vi "Calculate Vector Data.vi"(6 "Data In":T1, 8 "Display State In":T2 caption="State", 9 "X or Magnitude In":waveform(dbl), 10 "Y or Phase In":waveform(dbl), 11 "Order In":u16) -> (4 "Data Out":T1, 5 "R,Theta or X,Y Points Out":cluster{dbl, dbl}[](array[cluster]))   [LabVIEW 2012, in "Vector Function Generator.xctl"]
doc: "Based on the XControl's state, takes the two waveforms as eith R,theta or X,Y data and calculates a complex number waveform from the result/"
uses:
  Vector Function Generator.xctl
  Vector State.ctl
  Vector Data.ctl
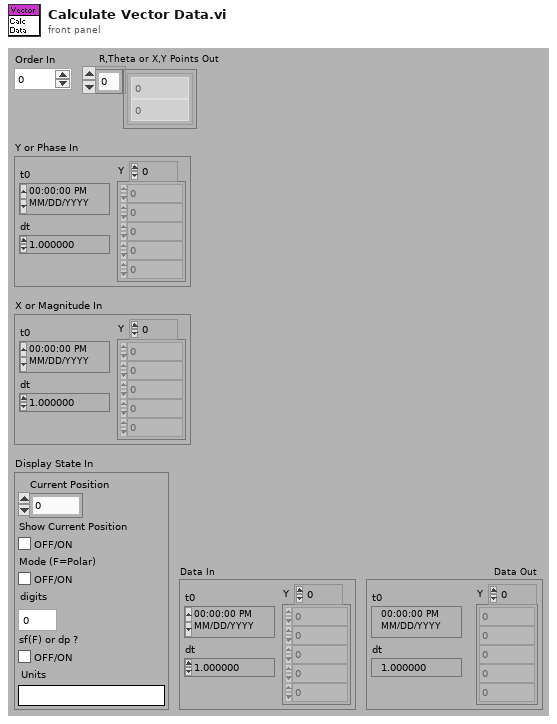
[diagram p1: front panel]
types:
  T1 = typedef "Vector Function Generator.xctl/Vector Data.ctl" = waveform(cdb)
  T2 = typedef "Vector Function Generator.xctl/Vector State.ctl" = cluster{"Current Position":i32, "Show Current Position":bool, "Mode (F=Polar)":bool, "digits":i32, "sf(F) or dp ?":bool, "Units":string}
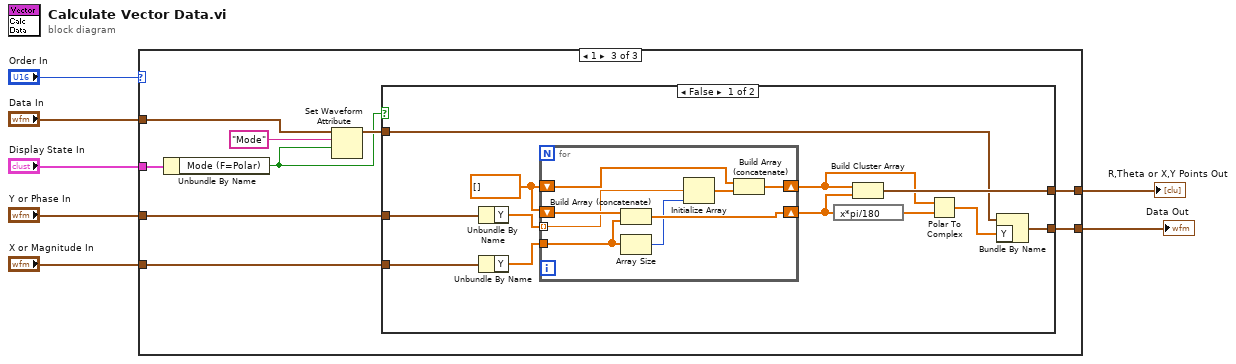
[diagram p0: block diagram]
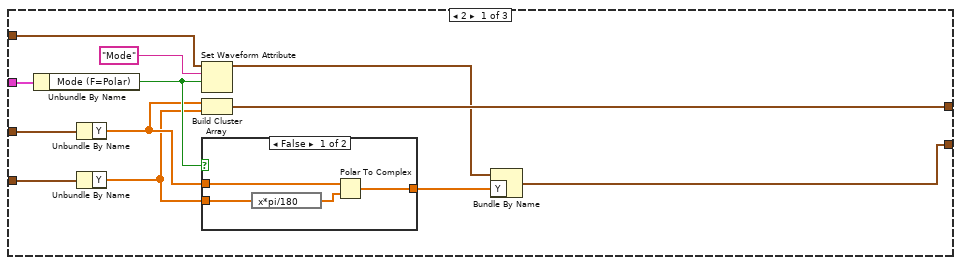
[diagram p2: hidden frame]
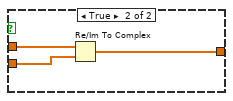
[diagram p3: hidden frame]
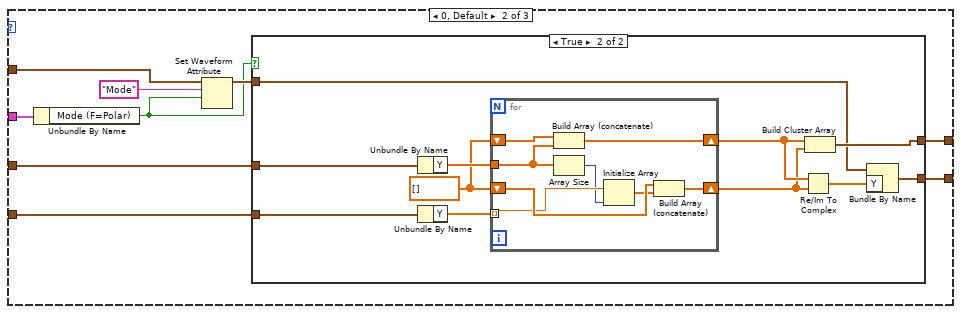
[diagram p4: hidden frame]
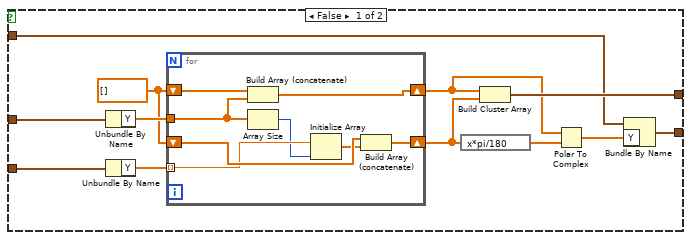
[diagram p5: hidden frame]
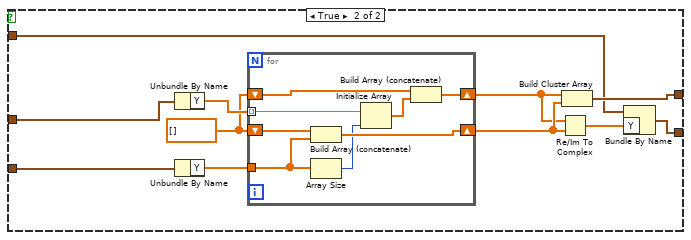
[diagram p6: hidden frame]
diagram:
  n1 = case shown="1" "Order In" {
    tunnel: [w19 w35 w83] -> w6
    tunnel: "Y or Phase In" -> [w18 w34 w82]
    tunnel: "X or Magnitude In" -> [w17 w31 w79]
    tunnel: "Data In" -> [w15 w32 w80]
    tunnel: [w12 w33 w81] -> w5
    tunnel: "Display State In" -> [w13 w30 w78]
    frame 2 {
      n2 = Unbundle By Name(w13) -> ("Mode (F=Polar)"=w11:bool)
      n3 = Unbundle By Name(w18) -> ("Y"=w10:dbl[])
      n4 = Unbundle By Name(w17) -> ("Y"=w9:dbl[])
      n5 = Set Waveform Attribute(5:w11, 6:"Mode" ("name"), 7:w15) -> (3:w14:T1)  [unwired: 1 in, 2 out]
      n6 = Build Cluster Array(w10, w9) -> (w19:cluster{dbl, dbl}[])
      n7 = case shown="False" w11 {
        tunnel: w10 -> [w23 w26]
        tunnel: w9 -> [w22 w25]
        tunnel: [w21 w24] -> w8
        frame False {
          n8 = expression code="x*pi/180"(w22) -> (w20:dbl[])
          n9 = Polar To Complex(1:w20, 2:w23) -> (0:w21:cdb[])
        }
        frame True {
          n10 = Re/Im To Complex(1:w25, 2:w26) -> (0:w24:cdb[])
        }
      }
      n11 = Bundle By Name(cluster=w14, "Y"=w8) -> (w12:T1)
    }
    frame 0, Default {
      n12 = Unbundle By Name(w30) -> ("Mode (F=Polar)"=w28:bool)
      n13 = Set Waveform Attribute(5:w28, 6:"Mode" ("name"), 7:w32) -> (3:w29:T1)  [unwired: 1 in, 2 out]
      n14 = case shown="True" w28 {
        tunnel: [w47 w66] -> w35
        tunnel: w34 -> [w46 w65]
        tunnel: [w38 w59] -> w33
        tunnel: w29 -> [w41 w63]
        tunnel: w31 -> [w43 w61]
        frame False {
          w44 = dbl[] []
          n15 = Unbundle By Name(w46) -> ("Y"=w45:dbl[])
          n16 = Unbundle By Name(w43) -> ("Y"=w42:dbl[])
          n17 = for {
            tunnel: w45 -> [w51]
            shift-right: [w55] -> w40
            shift-left: w44 -> [w54]
            shift-right: [w53] -> w37
            shift-left: w44 -> [w52]
            tunnel: w42 -> [w50] mode=indexing
            n18 = Build Array (concatenate)(w54, w51) -> (w55:dbl[])
            n19 = Array Size(array=w51) -> (size(s)=w49:i32)
            n20 = Initialize Array(w50, w49) -> (w48:dbl[])
            n21 = Build Array (concatenate)(w52, w48) -> (w53:dbl[])
          }
          n22 = expression code="x*pi/180"(w37) -> (w36:dbl[])
          n23 = Build Cluster Array(w40, w37) -> (w47:cluster{dbl, dbl}[])
          n24 = Polar To Complex(1:w36, 2:w40) -> (0:w39:cdb[])
          n25 = Bundle By Name(cluster=w41, "Y"=w39) -> (w38:T1)
        }
        frame True {
          w62 = dbl[] []
          n26 = Unbundle By Name(w65) -> ("Y"=w64:dbl[])
          n27 = Unbundle By Name(w61) -> ("Y"=w60:dbl[])
          n28 = for {
            tunnel: w64 -> [w70]
            shift-right: [w74] -> w58
            shift-left: w62 -> [w73]
            shift-right: [w72] -> w57
            shift-left: w62 -> [w71]
            tunnel: w60 -> [w69] mode=indexing
            n29 = Build Array (concatenate)(w73, w70) -> (w74:dbl[])
            n30 = Array Size(array=w70) -> (size(s)=w68:i32)
            n31 = Initialize Array(w69, w68) -> (w67:dbl[])
            n32 = Build Array (concatenate)(w71, w67) -> (w72:dbl[])
          }
          n33 = Re/Im To Complex(1:w57, 2:w58) -> (0:w56:cdb[])
          n34 = Build Cluster Array(w58, w57) -> (w66:cluster{dbl, dbl}[])
          n35 = Bundle By Name(cluster=w63, "Y"=w56) -> (w59:T1)
        }
      }
    }
    frame 1 {
      n36 = Unbundle By Name(w78) -> ("Mode (F=Polar)"=w76:bool)
      n37 = Set Waveform Attribute(5:w76, 6:"Mode" ("name"), 7:w80) -> (3:w77:T1)  [unwired: 1 in, 2 out]
      n38 = case shown="False" w76 {
        tunnel: [w95 w114] -> w83
        tunnel: w82 -> [w94 w113]
        tunnel: [w86 w107] -> w81
        tunnel: w77 -> [w92 w111]
        tunnel: w79 -> [w90 w109]
        frame False {
          w91 = dbl[] []
          n39 = Unbundle By Name(w94) -> ("Y"=w93:dbl[])
          n40 = Unbundle By Name(w90) -> ("Y"=w89:dbl[])
          n41 = for {
            tunnel: w93 -> [w98] mode=indexing
            shift-right: [w103] -> w88
            shift-left: w91 -> [w102]
            shift-right: [w101] -> w84
            shift-left: w91 -> [w100]
            tunnel: w89 -> [w96]
            n42 = Build Array (concatenate)(w100, w96) -> (w101:dbl[])
            n43 = Array Size(array=w96) -> (size(s)=w99:i32)
            n44 = Initialize Array(w98, w99) -> (w97:dbl[])
            n45 = Build Array (concatenate)(w102, w97) -> (w103:dbl[])
          }
          n46 = expression code="x*pi/180"(w84) -> (w85:dbl[])
          n47 = Build Cluster Array(w88, w84) -> (w95:cluster{dbl, dbl}[])
          n48 = Polar To Complex(1:w85, 2:w88) -> (0:w87:cdb[])
          n49 = Bundle By Name(cluster=w92, "Y"=w87) -> (w86:T1)
        }
        frame True {
          w110 = dbl[] []
          n50 = Unbundle By Name(w113) -> ("Y"=w112:dbl[])
          n51 = Unbundle By Name(w109) -> ("Y"=w108:dbl[])
          n52 = for {
            tunnel: w112 -> [w117] mode=indexing
            shift-right: [w122] -> w104
            shift-left: w110 -> [w121]
            shift-right: [w120] -> w105
            shift-left: w110 -> [w119]
            tunnel: w108 -> [w115]
            n53 = Build Array (concatenate)(w119, w115) -> (w120:dbl[])
            n54 = Array Size(array=w115) -> (size(s)=w118:i32)
            n55 = Initialize Array(w117, w118) -> (w116:dbl[])
            n56 = Build Array (concatenate)(w121, w116) -> (w122:dbl[])
          }
          n57 = Re/Im To Complex(1:w105, 2:w104) -> (0:w106:cdb[])
          n58 = Build Cluster Array(w104, w105) -> (w114:cluster{dbl, dbl}[])
          n59 = Bundle By Name(cluster=w111, "Y"=w106) -> (w107:T1)
        }
      }
    }
  }
  "R,Theta or X,Y Points Out" <- w6
  "Data Out" <- w5
